vi "Write Instrument.vi"(8 "error in (no error)":errorcluster, 10 "Instrument":T1, 11 "Submodule EOL configuration in":refnum<class "Submodule EOL configuration.lvclass">) -> (0 "error out":errorcluster, 3 "Submodule EOL configuration out":refnum<class "Submodule EOL configuration.lvclass">)   [LabVIEW 2025, in "Submodule EOL.lvlib" / "Submodule EOL configuration.lvclass"]
uses:
  Submodule EOL configuration.lvclass
  Instrumnet.ctl
  Submodule EOL configuration.lvclass/Submodule EOL configuration.ctl
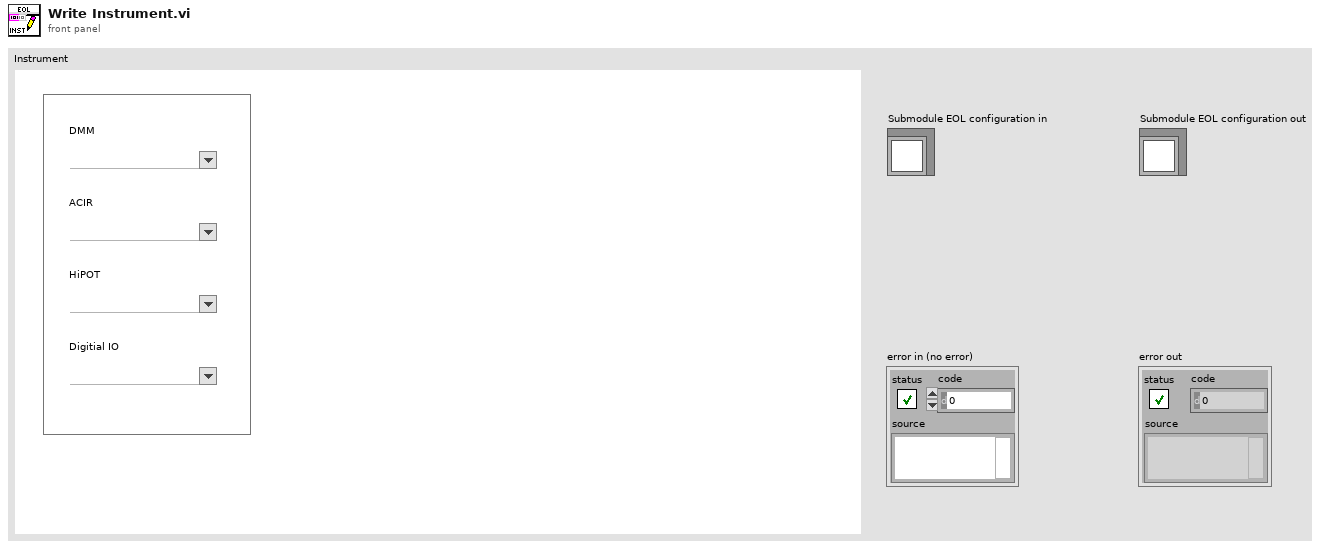
[diagram p1: front panel]
types:
  T1 = typedef "Submodule EOL.lvlib/Submodule EOL configuration.lvclass/Instrumnet.ctl" = cluster{"Digitial IO":string, "HiPOT":string, "ACIR":string, "DMM":string}
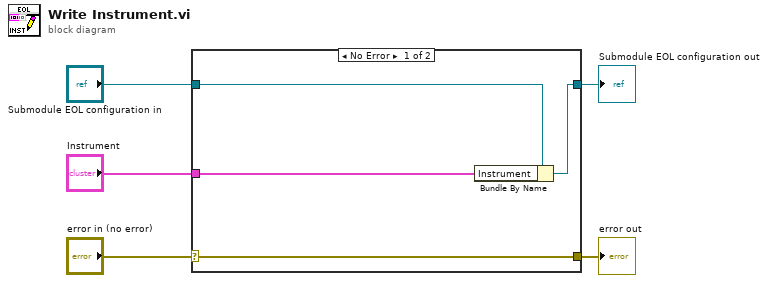
[diagram p0: block diagram]
diagram:
  n1 = case shown="No Error" "error in (no error)" {
    selector: "error in (no error)" -> [w9 w10]
    tunnel: [w9 w10] -> w4
    tunnel: [w7 w11] -> w2
    tunnel: "Submodule EOL configuration in" -> [w8 w11]
    tunnel: "Instrument" -> [w6 _]
    frame No Error {
      n2 = Bundle By Name(cluster=w8, "Instrument"=w6) -> (w7:refnum<class "Submodule EOL configuration.lvclass">)
    }
    frame Error {
    }
  }
  "error out" <- w4
  "Submodule EOL configuration out" <- w2
